vi "Initialize Tasks - NTask.vi"(6 "initialize and close session behavior":T1, 8 "error in":errorcluster, 11 "session reservation in":refnum<class "Session Reservation.lvclass">) -> (0 "error out":errorcluster, 1 "channel lists":string[](array[string]), 2 "tasks":refnum<class "Session Factory.lvclass">[](array[class]), 3 "session reservation out":refnum<class "Session Reservation.lvclass">)   [LabVIEW 2021, in "Session Management niDAQmx.lvlib"]
doc: "Creates the NI-DAQmx driver tasks from the <b>session reservation in</b>."
uses:
  Session Management niDAQmx.lvlib
  <vilib>/Plug-In SDKs/Clients/Session Management V1/Session Reservation/Initialize and Close Session Behavior.ctl
  <vilib>/Plug-In SDKs/Clients/Session Management V1/Session Reservation/Session Reservation.lvclass
  Session Factory/Session Factory.lvclass
  C:/Program Files/National Instruments/LabVIEW 2021/vi.lib/Plug-In SDKs/Sessions/Instrument/ISession Factory/ISession Factory.lvclass
  22e4e70a-b88f-404f-ac8b-cea03784f9c7.vi
  <vilib>/Plug-In SDKs/Clients/Session Management V1/Session Reservation/Initialize Sessions with Retry.vi
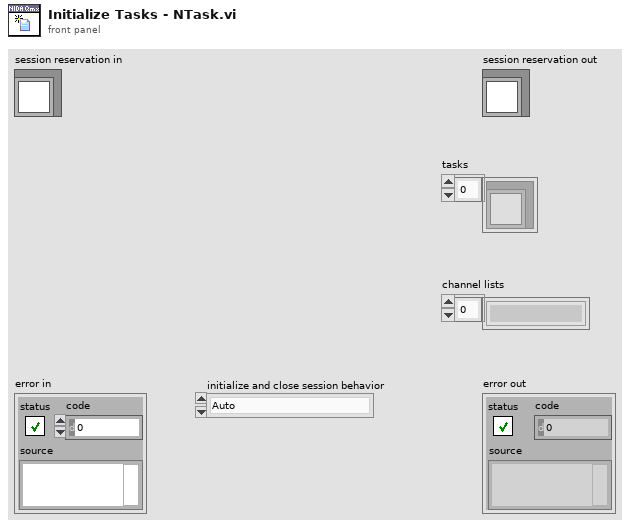
[diagram p1: front panel]
types:
  T1 = typedef "NI Session Management V1 Client.lvlib/Session Reservation.lvclass/Initialize and Close Session Behavior.ctl" = enum16{"Auto", "Initialize and Close", "Attach and Detach", "Initialize and Detach", "Attach and Close"}
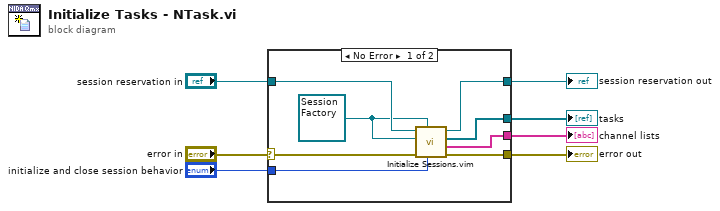
[diagram p0: block diagram]
diagram:
  n1 = case shown="No Error" "error in" {
    selector: "error in" -> [w15 w16]
    tunnel: "session reservation in" -> [w14 w17]
    tunnel: "initialize and close session behavior" -> [w13 _]
    tunnel: [w12 w16] -> w3
    tunnel: [w11 w17] -> w4
    tunnel: [w10 _] -> w1
    tunnel: [w9 _] -> w2
    frame No Error {
      w8 = refnum<class "Session Factory.lvclass"> refnum ("Session Management niDAQmx.lvlib:Session Factory.lvclass")
      n2 = call "Initialize Sessions.vim"("initialize and close session behavior"=w13, "session type"=w8, "error in"=w15, "session factory"=w8, "session reservation in"=w14) -> ("error out"=w12:errorcluster, "channel lists"=w9:string[], "sessions"=w10:refnum<class "Session Factory.lvclass">[], "session reservation out"=w11:refnum<class "Session Reservation.lvclass">)  [unwired: 3 in]
    }
    frame Error {
    }
  }
  "error out" <- w3
  "session reservation out" <- w4
  "channel lists" <- w2
  "tasks" <- w1
